vi "LoadGraphTxt (SubVI).vi"(11 "comm?":bool=TRUE) -> (3 "АЧХ":cluster{dbl[], dbl[]}[](graph) caption="XY Graph - Light")   [LabVIEW 2017]
panel:
  out "array w/ subset deleted":dbl[][](array[numeric])
  out "all rows":dbl[][](array[numeric])
  in  "error in":errorcluster
  out "error out":errorcluster
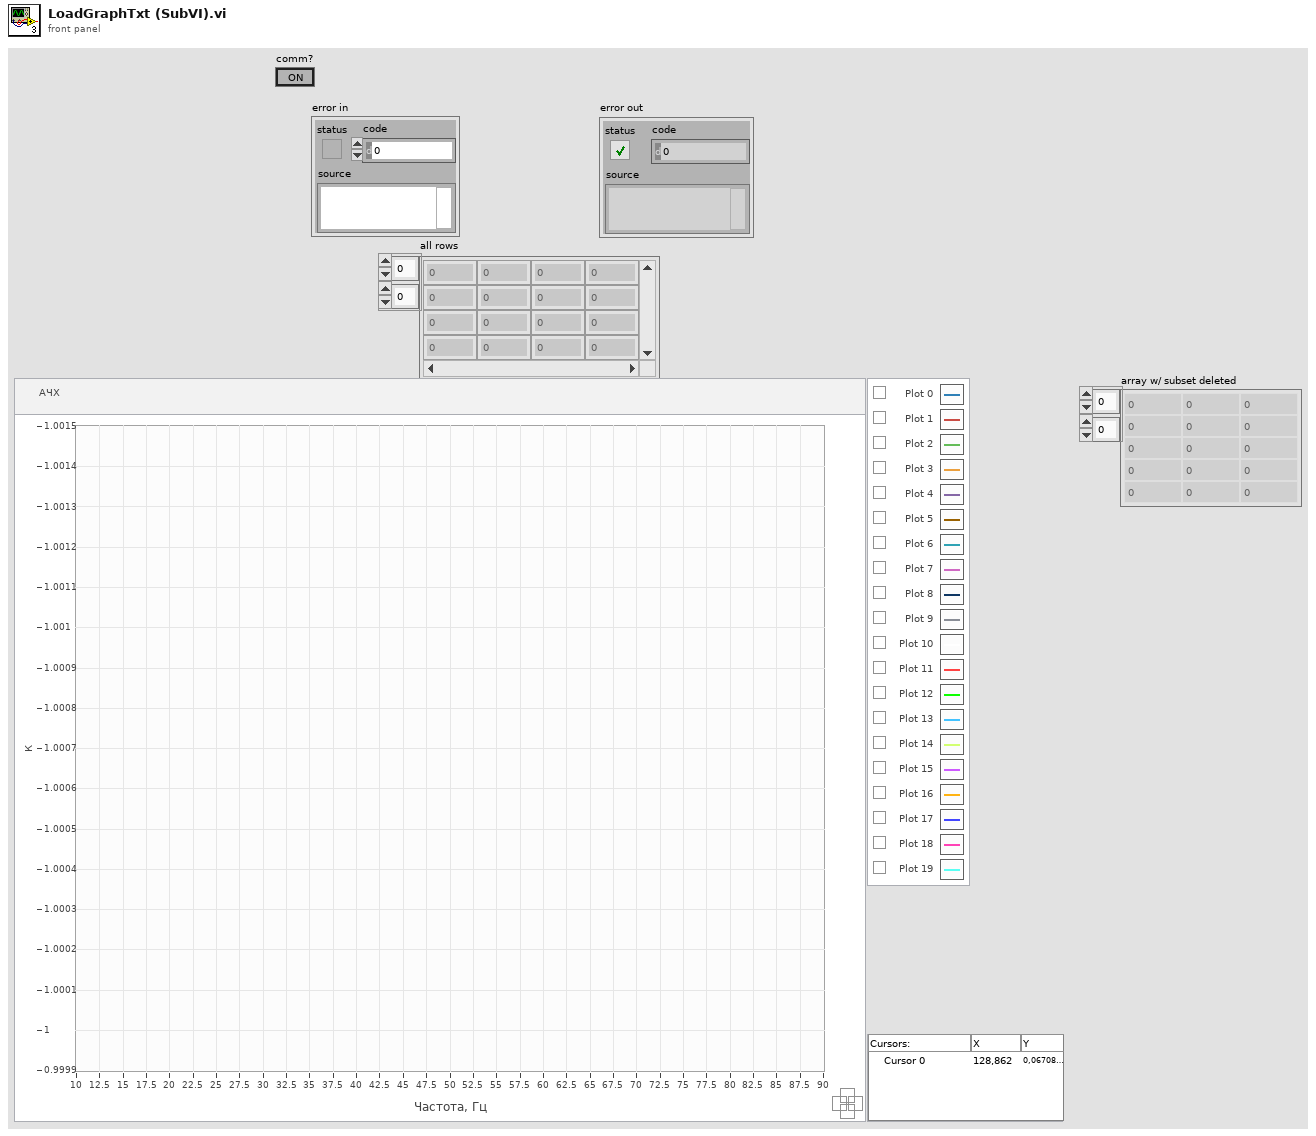
[diagram p1: front panel]
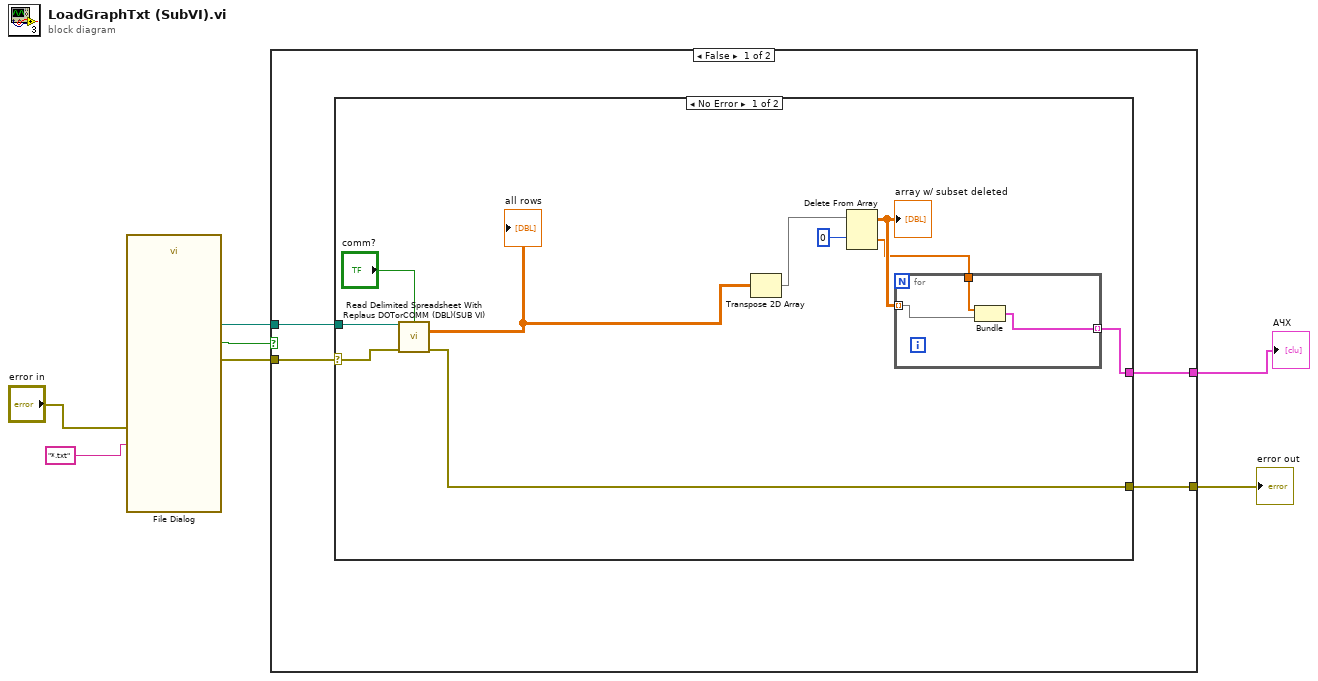
[diagram p0: block diagram]
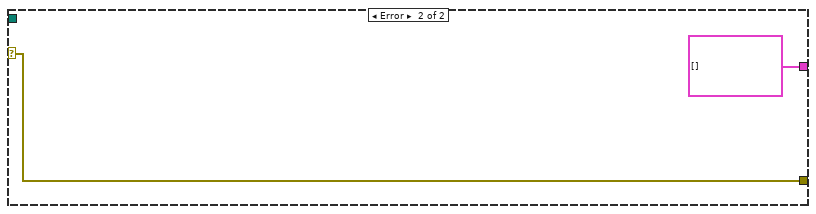
[diagram p2: hidden frame]
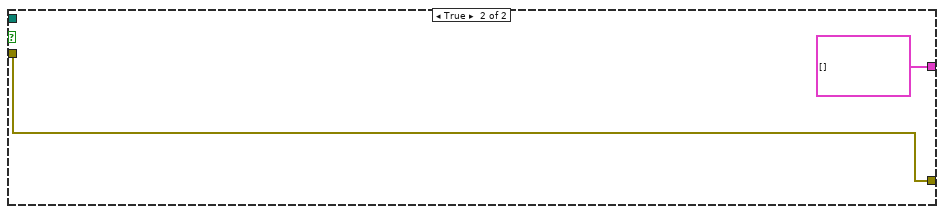
[diagram p3: hidden frame]
diagram:
  n1 = call "File Dialog"("error in"="error in", "pattern (all files)"="*.txt" ("default name")) -> ("selected path"=w7:path, "cancelled"=w4:bool, "error out"=w6:errorcluster)  [unwired: 10 in, 1 out]
  n2 = case shown="False" w4 {
    tunnel: w7 -> [w11 _]
    tunnel: w6 -> [w10 w28]
    tunnel: [w9 w28] -> w5
    tunnel: [w8 cluster{dbl[], dbl[]}[] [] ("appended array")] -> w1
    frame False {
      n3 = case shown="No Error" w10 {
        selector: w10 -> [w20 w26]
        tunnel: w11 -> [w21 _]
        tunnel: [w19 w26] -> w9
        tunnel: [w12 cluster{dbl[], dbl[]}[] [] ("appended array")] -> w8
        frame No Error {
          n4 = call "Read Delimited Spreadsheet With Replaus DOTorCOMM (DBL)(SUB VI).vi"("file path (dialog if empty)"=w21, "comm?"="comm?", "error in (no error)"=w20) -> ("all rows"=w17:dbl[][], "error out"=w19:errorcluster)  [unwired: 7 in, 4 out]
          "all rows" <- w17
          n5 = Transpose 2D Array(2D array=w17) -> (transposed array=w16:dbl[][])
          n6 = Delete From Array(array=w16, index (row)=0) -> (deleted portion=w13:dbl[], array with subset deleted=w14:dbl[][])  [unwired: 2 in]
          "array w/ subset deleted" <- w14
          n7 = for {
            tunnel: w14 -> [w24] mode=indexing
            tunnel: w13 -> [w23]
            tunnel: [w22] -> w12 mode=indexing
            n8 = Bundle(w23, w24) -> (w22:cluster{dbl[], dbl[]})  [unwired: 1 in]
          }
        }
        frame Error {
        }
      }
    }
    frame True {
    }
  }
  "error out" <- w5
  "АЧХ" <- w1
